vi "GetDIOConfiguration.vi"(8 "error in (no error)":errorcluster, 11 "DIO_Channel in":refnum<class "DIO_Channel.lvclass">) -> (0 "error out":errorcluster, 2 "Config":refnum<class "DIO-Configuration.lvclass">, 3 "DIO_Channel out":refnum<class "DIO_Channel.lvclass">)   [LabVIEW 2021, in "DIO-Channel.lvlib" / "DIO_Channel.lvclass"]
uses:
  DIO_Channel.lvclass
  C:/Users/averna/Documents/LV Gym DEMO/Factory Pattern/Generic Channel/Channel/Channel.lvclass
  DIO-Configuration_class/DIO-Configuration.lvclass
  Dependencies/Channel.lvlibp/Channel/Configuration_class/Configuration.lvclass
  DIO_Channel.lvclass/DIO_Channel.ctl
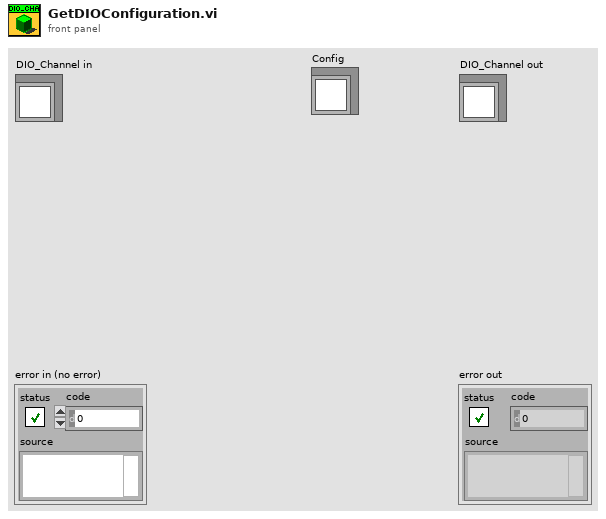
[diagram p1: front panel]
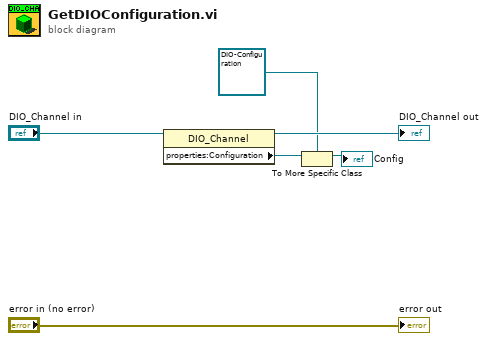
[diagram p0: block diagram]
diagram:
  n1 = property class="DIO_Channel"(reference="DIO_Channel in") -> (reference out=→"DIO_Channel out":refnum<class "DIO_Channel.lvclass">, "properties:Configuration"=w3:refnum<class "Configuration.lvclass">)  [unwired: 1 in, 1 out]
  n2 = To More Specific Class(target class=refnum<class "DIO-Configuration.lvclass"> refnum ("DIO-Channel.lvlib:DIO_CFG"), reference=w3) -> (specific class reference=→"Config":refnum<class "DIO-Configuration.lvclass">)  [unwired: 1 in, 1 out]
  "error out" <- "error in (no error)"
